vi "Add to Sector Accumulation.vi"(6 "Pixel y":u16, 7 "Pixel x":u16, 9 "[Accumulated Sectors] In":T2[](array[typedef]), 10 "Pixel Intensity":u8, 11 "Sector ID":u8) -> (2 "Sector Pixel":T1, 3 "[Accumulated Sectors] Out":T2[](array[typedef]))   [LabVIEW 2013]
uses:
  FPGA/Sector/Accumulate/Accumulated Sector Cluster.ctl
  Test Compiliation/Test Sector Cluster.ctl
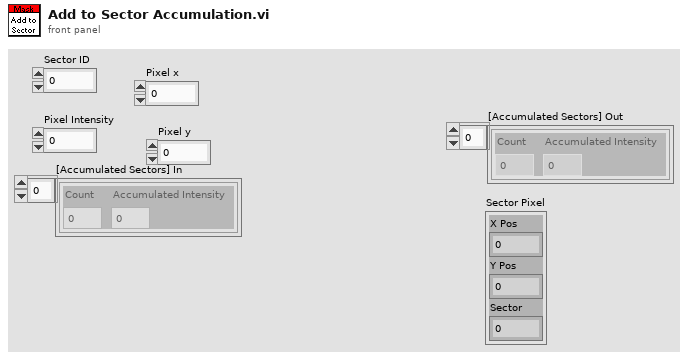
[diagram p1: front panel]
types:
  T1 = typedef "Test Sector Cluster.ctl" = cluster{"X Pos":u16, "Y Pos":u16, "Sector":u8}
  T2 = typedef "Accumulated Sector Cluster.ctl" = cluster{"Accumulated Intensity":u32, "Count":u16}
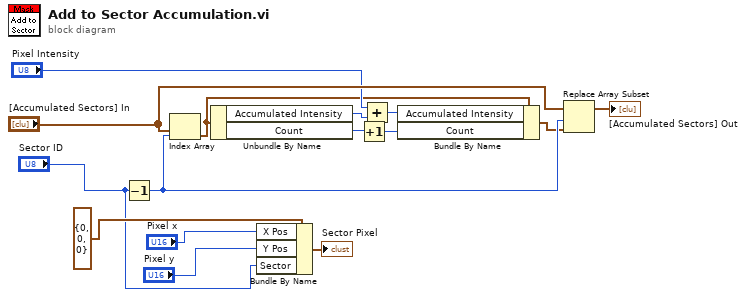
[diagram p0: block diagram]
diagram:
  n1 = Decrement(x="Sector ID") -> (x-1=w11:u8)
  n2 = Index Array(array="[Accumulated Sectors] In", index=w11) -> (element=w7:T2)
  n3 = Unbundle By Name(w7) -> ("Accumulated Intensity"=w13:u32, "Count"=w15:u16)
  n4 = Bundle By Name(cluster=T1 {"X Pos"=0, "Y Pos"=0, "Sector"=0} ("Test Sector"), "X Pos"="Pixel x", "Y Pos"="Pixel y", "Sector"="Sector ID") -> (→"Sector Pixel":T1)
  n5 = Increment(x=w15) -> (x+1=w14:u16)
  n6 = Add(x="Pixel Intensity", y=w13) -> (x+y=w12:u32)
  n7 = Bundle By Name(cluster=w7, "Accumulated Intensity"=w12, "Count"=w14) -> (w6:T2)
  n8 = Replace Array Subset(array="[Accumulated Sectors] In", new element=w6, index=w11) -> (→"[Accumulated Sectors] Out":T2[])
